vi "REP-REQ TCP.vi"(7 "TcpRouter-Client in":refnum<class "TcpRouter-Client.lvclass">, 8 "error in (no error)":errorcluster, 9 "timeout ms (minus value for input)":i32) -> (0 "error out":errorcluster, 2 "REQ-REP":refnum<data-value>, 3 "connection ID":refnum<k5>)   [LabVIEW 2020, in "CSM-TCP-Router.lvlib" / "TcpRouter-Client.lvclass"]
uses:
  TcpRouter-Client.lvclass
  Def-TCP-Router REQ-REP.ctl
  TcpRouter-Client.lvclass/TcpRouter-Client.ctl
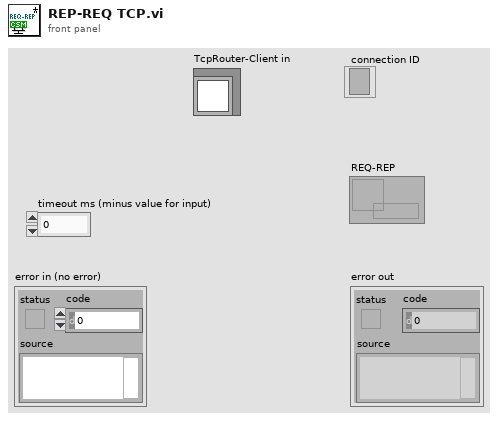
[diagram p1: front panel]
types:
  T1 = cluster{"IP Address":string, "Port":u16, "ConnectTMO":i32}
  T2 = typedef "CSM-TCP-Router.lvlib/TcpRouter-Client.lvclass/Def-TCP-Router REQ-REP.ctl" = cluster{"REQ-REP":refnum<k5>}
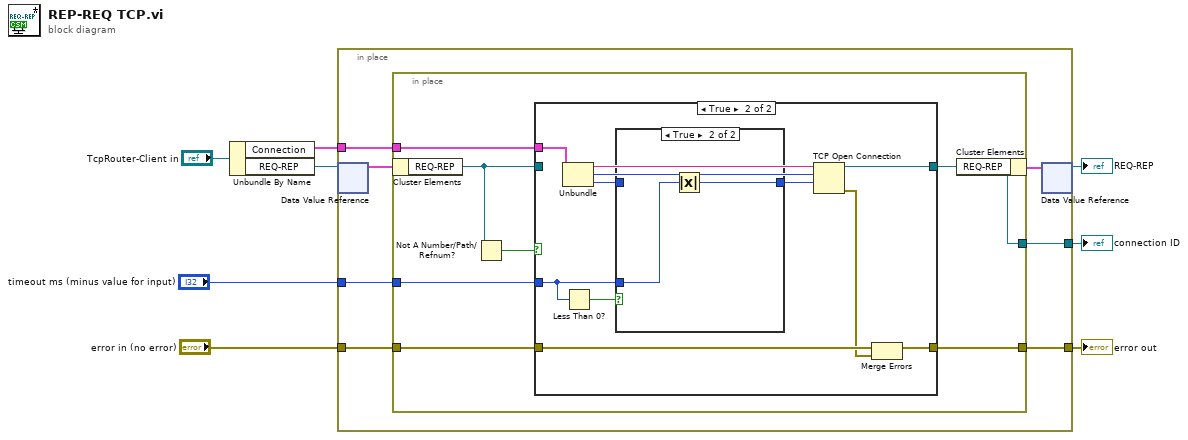
[diagram p0: block diagram]
diagram:
  n1 = Unbundle By Name("TcpRouter-Client in") -> ("Connection"=w4:T1, "REQ-REP"=w5:refnum<data-value>)
  n2 = in-place {
    in-place-border: w4 -> [w13]
    in-place-border: [w12] -> w7
    in-place-border: "error in (no error)" -> [w11]
    in-place-border: [w10] -> w3
    in-place-border: "timeout ms (minus value for input)" -> [w9]
    n3 = in-place-dvr #1(w5) -> (w15:T2)  [unwired: 1 out]
    n4 = in-place {
      in-place-border: w13 -> [w22]
      in-place-border: [w20] -> w12
      in-place-border: w11 -> [w21]
      in-place-border: [w17] -> w10
      in-place-border: w9 -> [w16]
      n5 = in-place-cluster #2(w15) -> ("REQ-REP"=w18:refnum<k5>)
      n6 = Not A Number/Path/Refnum?(number/path/refnum=w18) -> (NaN/Path/Refnum?=w19:bool)
      n7 = case shown="True" w19 {
        tunnel: w22 -> [_ w33]
        tunnel: w21 -> [w23 w32]
        tunnel: [w23 w31] -> w20
        tunnel: [w24 w29] -> w17
        tunnel: w18 -> [w24 _]
        tunnel: w16 -> [_ w26]
        frame False {
        }
        frame True {
          n8 = Unbundle(w33) -> ("IP Address"=w35:string, "Port"=w34:u16, "ConnectTMO"=w27:i32)
          n9 = Less Than 0?(x=w26) -> (x < 0?=w25:bool)
          n10 = case shown="True" w25 {
            tunnel: [w36 w37] -> w28
            tunnel: w27 -> [w36 _]
            tunnel: w26 -> [_ w38]
            frame False {
            }
            frame True {
              n11 = Absolute Value(x=w38) -> (abs(x)=w37:i32)
            }
          }
          n12 = TCP Open Connection(address=w35, remote port or service name=w34, timeout ms (60000)=w28) -> (connection ID=w29:refnum<k5>, error out=w30:errorcluster)  [unwired: 2 in]
          n13 = Merge Errors(w32, w30) -> (w31:errorcluster)
        }
      }
      n14 = in-place-cluster #2("REQ-REP"=w17) -> (w14:T2)
    }
    n15 = in-place-dvr #1(w14) -> (→"REQ-REP":refnum<data-value>)  [unwired: 1 out]
  }
  "error out" <- w7
  "connection ID" <- w3
